vi "Sous_VI_Virage_1.vi"(8 "error in (no error)":errorcluster) -> (0 "error out":errorcluster)   [LabVIEW 2017]
panel:
  out "x > y ? 3":bool[](array[boolean])
  out "x > y ? 2":bool[](array[boolean])
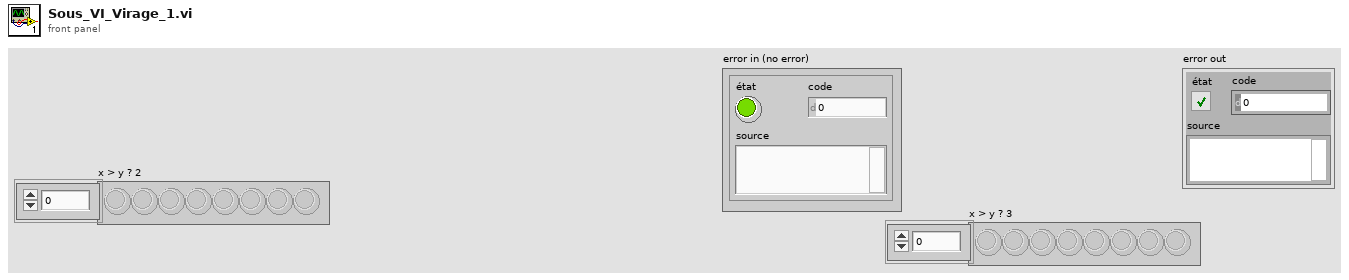
[diagram p1: front panel]
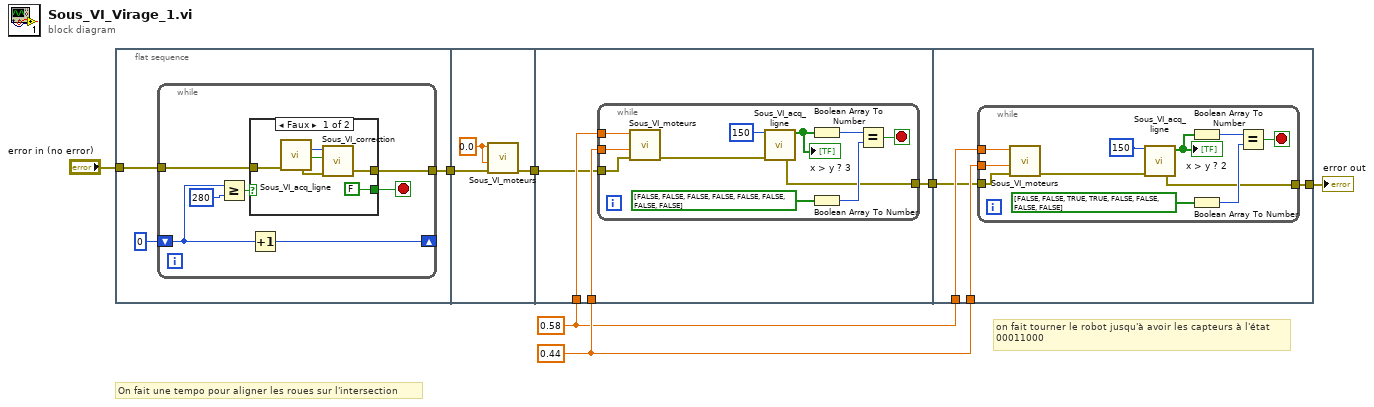
[diagram p0: block diagram]
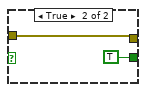
[diagram p2: hidden frame]
diagram:
  w6 = 0.58 ("moteur gauche vite")
  w7 = 0.44 ("moteur droit lent")
  # "on fait tourner le robot jusqu'à avoir les capteurs à l'état\n00011000"
  # "On fait une tempo pour aligner les roues sur l'intersection"
  n1 = flat-sequence {
    tunnel: "error in (no error)" -> [w9]
    tunnel: [w8] -> w4
    tunnel: w4 -> [w27]
    tunnel: [w26] -> w3
    tunnel: w7 -> [w31]
    tunnel: w6 -> [w32]
    tunnel: w3 -> [w30]
    tunnel: [w29] -> w2
    tunnel: w6 -> [w47]
    tunnel: w7 -> [w46]
    tunnel: w2 -> [w45]
    tunnel: [w44] -> w1
    frame #0 {
      n2 = while {
        shift-right: [w17] -> _
        shift-left: 0 -> [w14]
        tunnel: w9 -> [w12]
        tunnel: [w11] -> w8
        stop <- w15 stop-if-true
        n3 = Greater Or Equal?(x=w14, y=280) -> (x >= y?=w16:bool)
        n4 = case shown="Faux" w16 {
          tunnel: [FALSE TRUE] -> w15
          tunnel: w12 -> [w20 w24]
          tunnel: [w18 w24] -> w11
          frame False {
            n5 = call "Sous_VI_acq_ligne.vi"("error in (no error)"=w20) -> ("Décalage"=w22:u32, "G/D ?"=w21:bool, "error out"=w19:errorcluster)  [unwired: 9 in, 3 out]
            n6 = call "Sous_VI_correction.vi"("error in (no error)"=w19, "G/D ?"=w21, "Décalage"=w22) -> ("error out"=w18:errorcluster)  [unwired: 8 in]
          }
          frame True {
          }
        }
        n7 = Increment(x=w14) -> (x+1=w17:i32)
      }
    }
    frame #1 {
      w28 = 0.0 ("Moteur Gauche")
      n8 = call "Sous_VI_moteurs.vi"("error in (no error)"=w27, "Moteur Droit"=w28, "Moteur Gauche"=w28) -> ("error out"=w26:errorcluster)  [unwired: 8 in]
    }
    frame #2 {
      n9 = while {
        tunnel: w32 -> [w39]
        tunnel: w31 -> [w36]
        tunnel: w30 -> [w35]
        tunnel: [w33] -> w29
        stop <- w40 stop-if-true
        n10 = call "Sous_VI_moteurs.vi"("error in (no error)"=w35, "Moteur Droit"=w36, "Moteur Gauche"=w39) -> ("error out"=w34:errorcluster)  [unwired: 8 in]
        n11 = call "Sous_VI_acq_ligne.vi"("Seuil"=150, "error in (no error)"=w34) -> ("x > y ?"=w38:bool[], "error out"=w33:errorcluster)  [unwired: 8 in, 4 out]
        "x > y ? 3" <- w38
        n12 = Boolean Array To Number(Boolean array=w38) -> (number=w41:u32)
        n13 = Boolean Array To Number(Boolean array=bool[] [FALSE, FALSE, FALSE, FALSE, FALSE, FALSE, FALSE, FALSE]) -> (number=w42:u32)
        n14 = Equal?(x=w41, y=w42) -> (x = y?=w40:bool)
      }
    }
    frame #3 {
      n15 = while {
        tunnel: w47 -> [w54]
        tunnel: w46 -> [w51]
        tunnel: w45 -> [w50]
        tunnel: [w48] -> w44
        stop <- w55 stop-if-true
        n16 = call "Sous_VI_moteurs.vi"("error in (no error)"=w50, "Moteur Droit"=w51, "Moteur Gauche"=w54) -> ("error out"=w49:errorcluster)  [unwired: 8 in]
        n17 = call "Sous_VI_acq_ligne.vi"("Seuil"=150, "error in (no error)"=w49) -> ("x > y ?"=w53:bool[], "error out"=w48:errorcluster)  [unwired: 8 in, 4 out]
        "x > y ? 2" <- w53
        n18 = Boolean Array To Number(Boolean array=w53) -> (number=w56:u32)
        n19 = Boolean Array To Number(Boolean array=bool[] [FALSE, FALSE, TRUE, TRUE, FALSE, FALSE, FALSE, FALSE]) -> (number=w57:u32)
        n20 = Equal?(x=w56, y=w57) -> (x = y?=w55:bool)
      }
    }
  }
  "error out" <- w1
